vi "VTU_Reference_Load_Calc.vi"(8 "error in (no error)":errorcluster={"status"=FALSE, "code"=0, "source"="\"\""}, 10 "delta_mm":dbl=2.0, 11 "base_stroke_mm":dbl=10.0) -> (0 "error out":errorcluster={"status"=FALSE, "code"=0, "source"="\"\""}, 3 "computed_target_mm":dbl)   [LabVIEW 2026]
doc: "INTENT: Dynamic VTU hydraulic load calculation from measured stroke and relative displacement."
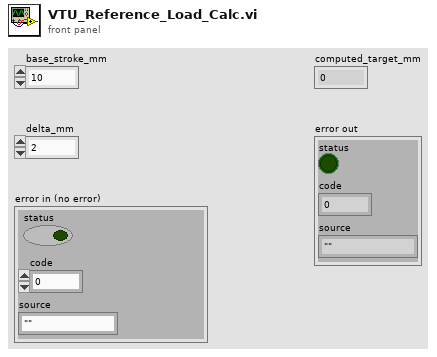
[diagram p1: front panel]
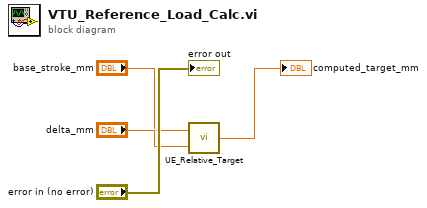
[diagram p0: block diagram]
diagram:
  n1 = call "UE_Relative_Target.vi"("offset_mm"="delta_mm", "reference_mm"="base_stroke_mm") -> ("target_mm"=→"computed_target_mm":dbl)
  "error out" <- "error in (no error)"
